vi "U8 Performance Test.vi"() -> ()   [LabVIEW 2021]
uses:
  ChannelCommon/typedef/Benchmark Stats.ctl
  ChannelCommon/typedef/Direction.ctl
  CIF_Iceoryx_PCAP_Universal.lvclass
  D:/dev/Packages/CIF_Channels_Core/src/CIFChannels/CIFChannels.lvclass
  Iceorxy Utilities/Typedef/PCAP Config.ctl
  ChannelCommon/typedef/New FIFO Config.ctl
  ChannelCommon/typedef/FIFO Flags.ctl
  Iceorxy Utilities/Typedef/PCAP Linktype.ctl
  ChannelCommon/typedef/New FIFO Instance Configuration.ctl
  <vilib>/Platform/TimedLoop/XDataNode/timing_clust.ctl
  <vilib>/Platform/TimedLoop/XDataNode/nitl_modes.ctl
  <vilib>/Platform/TimedLoop/XDataNode/wakeup.ctl
  ChannelCommon/typedef/TimeStamps.ctl
  CIFChannels/CIFChannels.lvclass/CIFChannels.ctl
  <vilib>/CIF Foundation/CIF Utilities/Statistics/I64/Stats_I64_CIF_U.lvclass/Stats_I64_CIF_U.ctl
  <vilib>/CIF Foundation/CIF Utilities/Statistics/I64/Get Stats.vi
  <vilib>/Platform/TimedLoop/XDataNode/XDataNode.xnode
  <vilib>/Platform/TimedLoop/XDataNode/XDNodeRunTimeDep.lvlib
  ChannelCommon/ChannelCommon.lvlib
  CIFChannels/CIFChannels.lvclass
  Iceorxy Utilities/Iceoryx Channel Utilities.lvlib
panel:
  in  "stop":bool
  out "Flatten (us) TO":T1
  out "Channel R/W (us) TO":T1
  out "Flatten (us)":T1
  out "Channel R/W (us)":T1
  out "avg TO":dbl
  out "max TO":dbl
  out "timed out? 3":bool
  out "timed out?":bool
  out "avg channel":dbl
  out "max channel":dbl
  out "pass":bool
  out "error out":errorcluster
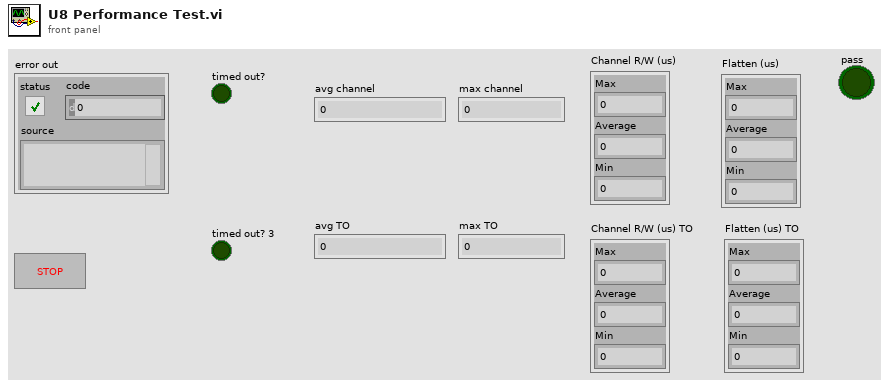
[diagram p1: front panel]
types:
  T1 = typedef "ChannelCommon.lvlib/Benchmark Stats.ctl" = cluster{"Max":i64, "Average":dbl, "Min":i64}
  T2 = typedef "Iceoryx Channel Utilities.lvlib/PCAP Config.ctl" = cluster{"New FIFO Config":T3, "Linktype":T5, "Linktype Override":u32, "Type Name Override":string}
  T3 = typedef "ChannelCommon.lvlib/New FIFO Config.ctl" = cluster{"Max Bytes/Msg":u64, "Max Msg/FIFO":u64, "FIFO Flags":T4, "Best Effort Subscribers":u32, "Backpressure Subscribers":u32}
  T4 = typedef "ChannelCommon.lvlib/FIFO Flags.ctl" = cluster{"Backpressure":bool, "Extended Config":bool}
  T5 = typedef "Iceoryx Channel Utilities.lvlib/PCAP Linktype.ctl" = u32
  T6 = typedef "ChannelCommon.lvlib/Direction.ctl" = enum8{"Publisher", "Subscriber"}
  T7 = typedef "ChannelCommon.lvlib/New FIFO Instance Configuration.ctl" = cluster{"Backpressure":bool, "Bytes/Message Override":u32, "Messages/FIFO Override":u32, "Custom Data":u8[]}
  T8 = typedef "ChannelCommon.lvlib/TimeStamps.ctl" = cluster{"ClockID":u8, "T0":i64, "T_Out":i64}
  T9 = typedef "XDNodeRunTimeDep.lvlib/timing_clust.ctl" = cluster{"Expected End [f-1]":u64, "Actual End [f-1]":u64, "Finished Late? [f-1]":bool, "Expected End [i-1]":u64, "Actual End [i-1]":u64, "Finished Late? [i-1]":bool, "Expected Start [i]":u64, "Actual Start [i]":u64, "Expected Start [f]":u64, "Actual Start [f]":u64, "Source Name":string, "Structure Name":string, "Period":i64, "Deadline":i64, "Offset":i64, "Start":i64, "Priority":i32, "Timeout":i32, "Mode":T10, "Wakeup Reason":T11, "Error":errorcluster, "Source Type":string, "Secondary Source Type":string, "Global End Time":u64, "Global Start Time":u64, "Frame Duration":u64, "Iteration Duration":u64, "Assigned CPU":i32, "I/O Scan Engine Mode":u32}
  T10 = typedef "XDNodeRunTimeDep.lvlib/nitl_modes.ctl" = enum32{"No Change", "Process missed periods, maintain original phase", "Discard missed periods, maintain original phase", "Process missed periods, ignore original phase", "Discard missed periods, ignore original phase"}
  T11 = typedef "XDNodeRunTimeDep.lvlib/wakeup.ctl" = enum32{"Normal", "Aborted", "Asynchronous wakeup", "Timing source error", "Timed loop error", "Timeout"}
  T12 = typedef "ChannelCommon.lvlib/New FIFO Instance Response.ctl" = cluster{"Publisher":string, "Custom Data":u8[]}
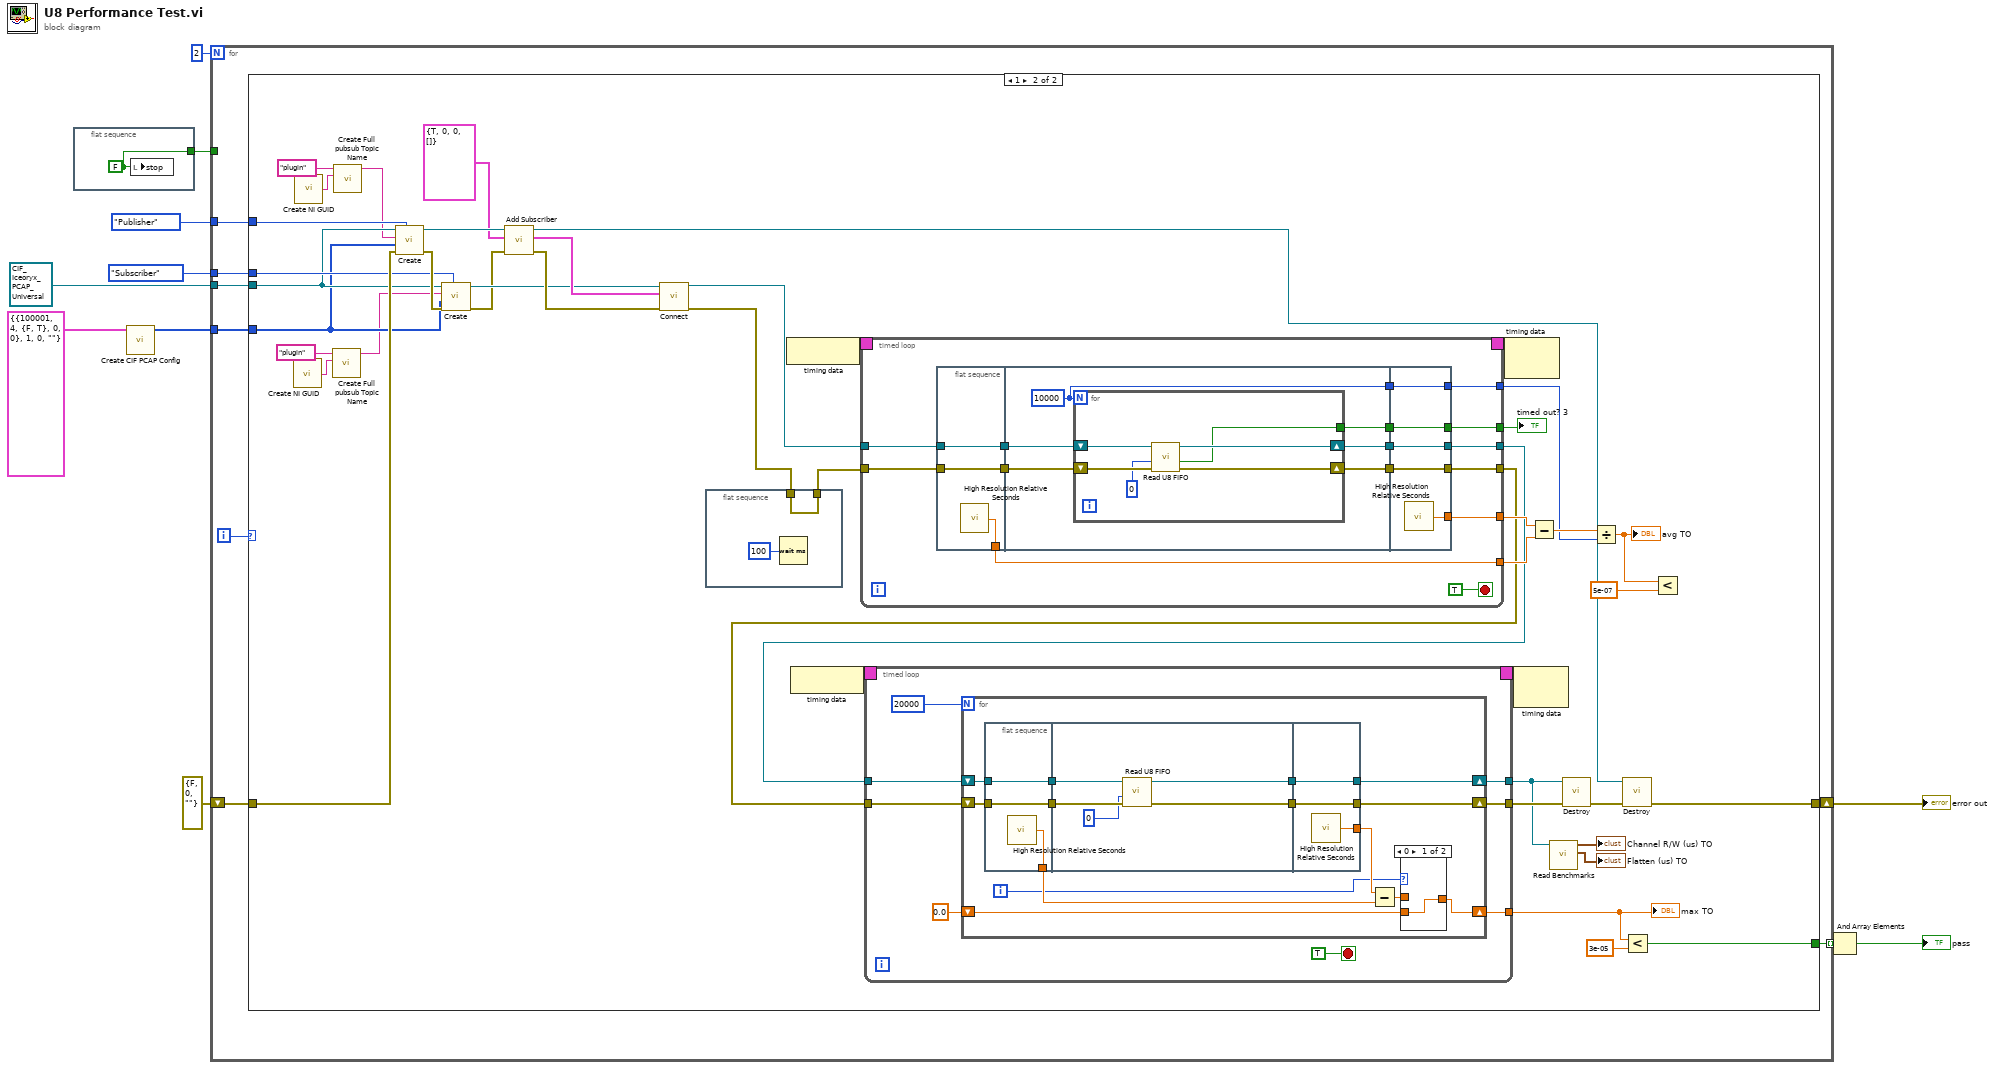
[diagram p0: block diagram]
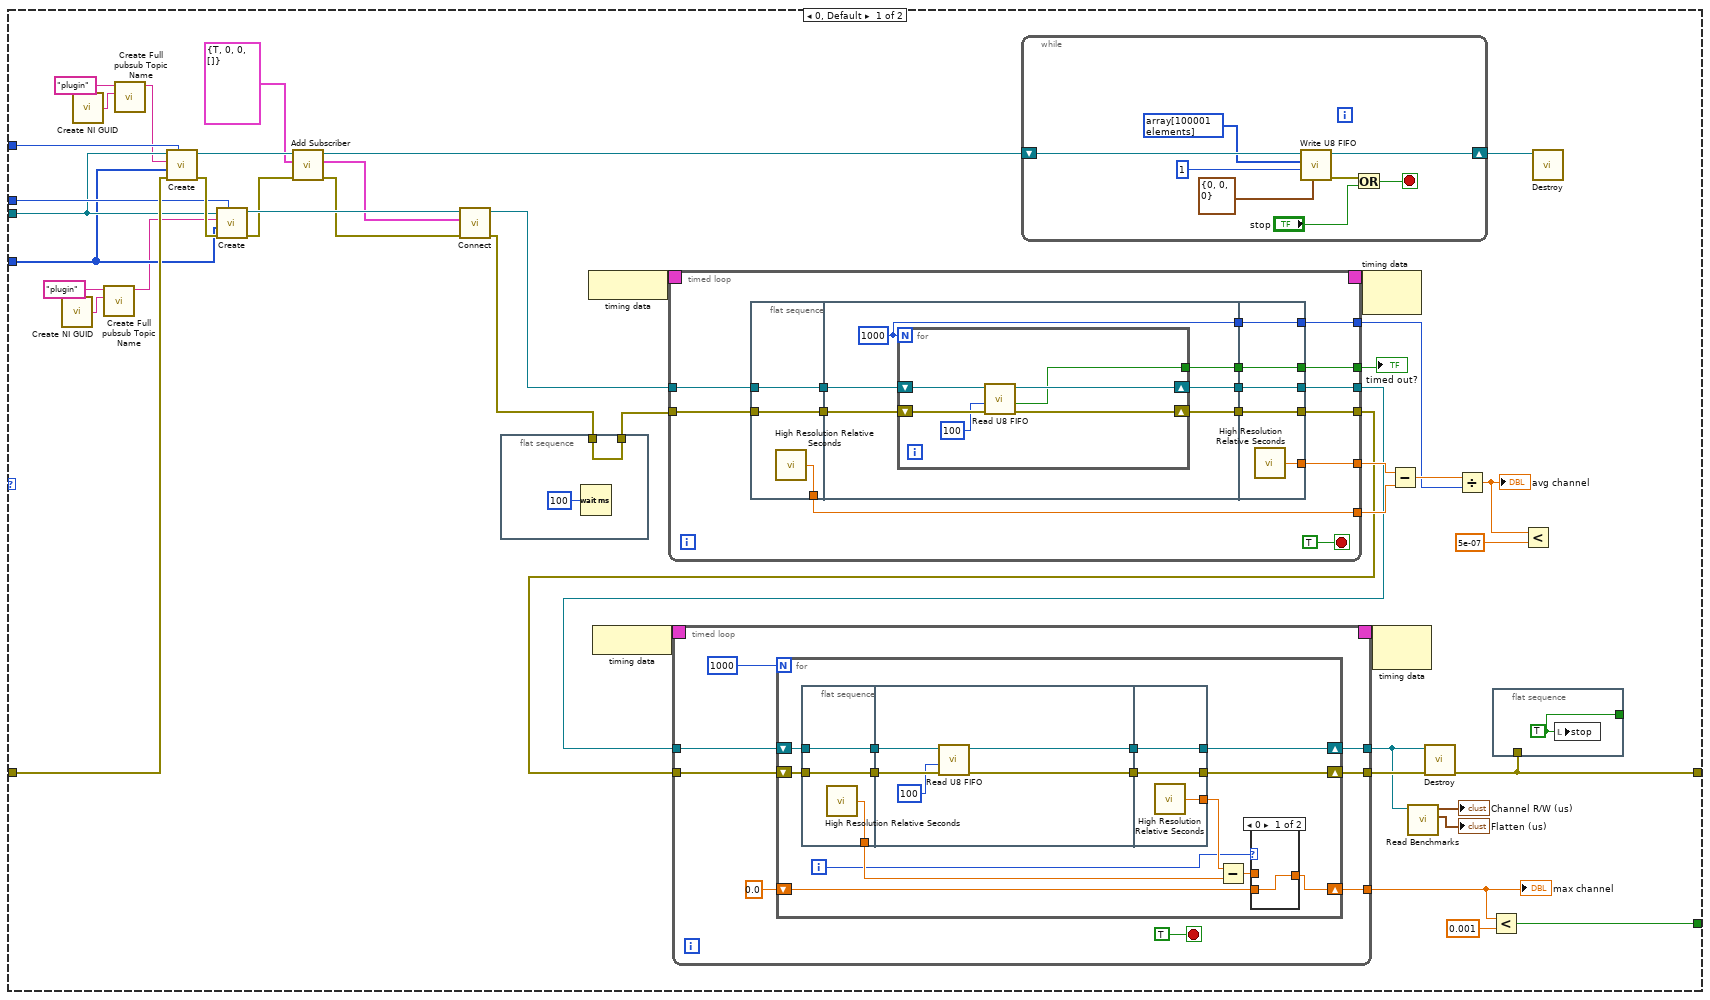
[diagram p2: hidden frame]
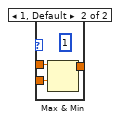
[diagram p3: hidden frame]
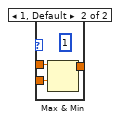
[diagram p4: hidden frame]
diagram:
  n1 = flat-sequence {
    tunnel: [w12] -> w3
    frame #0 {
      w12 = FALSE ("stop")
      n2 = local write "stop"(w12) -> ()
    }
  }
  n3 = call "Create CIF PCAP Config.vi"("PCAP FIFO Config"=T2 {"New FIFO Config"={"Max Bytes/Msg"=100001, "Max Msg/FIFO"=4, "FIFO Flags"={"Backpressure"=FALSE, "Extended Config"=TRUE}, "Best Effort Subscribers"=0, "Backpressure Subscribers"=0}, "Linktype"=1, "Linktype Override"=0, "Type Name Override"=""}) -> ("Flattened PCAP FIFO Config"=w1:u8[])  [unwired: 10 in]
  n4 = for {
    N: 2 -> [_]
    tunnel: [w20] -> w9 mode=indexing
    shift-right: [w19] -> w11
    shift-left: errorcluster {"status"=FALSE, "code"=0, "source"=""} ("error out") -> [w17]
    tunnel: Direction."Publisher" ("Direction") -> [w16]
    tunnel: Direction."Subscriber" ("Direction") -> [w15]
    tunnel: refnum<class "CIF_Iceoryx_PCAP_Universal.lvclass"> refnum ("CIF_CIPC_Fifo_U8.lvclass") -> [w14]
    tunnel: w1 -> [w13]
    tunnel: w3 -> [_]
    i -> [w18]
    n5 = case shown="1" w18 {
      tunnel: [w50 w185] -> w20
      tunnel: [w33 w176] -> w19
      tunnel: w17 -> [w48 w183]
      tunnel: w16 -> [w47 w182]
      tunnel: w15 -> [w46 w181]
      tunnel: w14 -> [w45 w180]
      tunnel: w13 -> [w43 w179]
      frame 0, Default {
        n6 = call <vilib>:"Create NI GUID.vi"() -> ("NI GUID"=w22:string)
        n7 = call <vilib>:"Create NI GUID.vi"() -> ("NI GUID"=w26:string)
        n8 = call "Create Full pubsub Topic Name.vi"("Topic"=w22, "Plugin name"="plugin") -> ("Full Topic"=w21:string)  [unwired: 8 in, 1 out]
        n9 = call "Create Full pubsub Topic Name.vi"("Topic"=w26, "Plugin name"="plugin") -> ("Full Topic"=w24:string)  [unwired: 8 in, 1 out]
        n10 = call-dynamic "Create.vi"("Direction"=w47, "error in (no error)"=w48, "Custom Config Data"=w43, "Name"=w24, "CIFFIFO in"=w45) -> ("error out"=w49:errorcluster, "CIFFIFO out"=w32:refnum<class "CIF_Iceoryx_PCAP_Universal.lvclass">)  [unwired: 5 in]
        n11 = call-dynamic "Create.vi"("Direction"=w46, "error in (no error)"=w49, "Custom Config Data"=w43, "Name"=w21, "CIFFIFO in"=w45) -> ("error out"=w30:errorcluster, "CIFFIFO out"=w44:refnum<class "CIF_Iceoryx_PCAP_Universal.lvclass">)  [unwired: 5 in]
        n12 = call-dynamic "Add Subscriber.vi"("error in (no error)"=w30, "New FIFO Instance Config"=T7 {"Backpressure"=TRUE, "Bytes/Message Override"=0, "Messages/FIFO Override"=0, "Custom Data"=[]}, "CIF_CIPC_Chn in"=w32) -> ("error out"=w29:errorcluster, "New FIFO Instance"=w28:T12, "CIF_CIPC_Chn out"=w31:refnum<class "CIF_Iceoryx_PCAP_Universal.lvclass">)  [unwired: 6 in]
        n13 = call-dynamic "Connect.vi"("error in (no error)"=w29, "Connection"=w28, "CIF_Iceoryx_PCAP"=w44) -> ("error out"=w40:errorcluster, "CIF_Iceoryx_PCAP"=w42:refnum<class "CIF_Iceoryx_PCAP_Universal.lvclass">)  [unwired: 7 in]
        n14 = flat-sequence {
          tunnel: w40 -> [w67]
          tunnel: [w67] -> w39
          frame #0 {
            n15 = Wait (ms)(milliseconds to wait=u32 100) -> ()  [unwired: 1 out]
          }
        }
        n16 = node-c288() -> (w64:T9)
        n17 = node-c288() -> (w62:T9)
        n18 = timed-loop {
          timing: w64 -> [_]
          timing-out: [_] -> w63
          tunnel: w42 -> [w131]
          tunnel: w39 -> [w130]
          tunnel: [w126] -> w56
          tunnel: [w124] -> w55
          tunnel: [w122] -> w60
          tunnel: [w121] -> w59
          tunnel: [w120] -> w57
          tunnel: [w118] -> w38
          stop <- TRUE stop-if-true
          n19 = flat-sequence {
            tunnel: w130 -> [w133]
            tunnel: w131 -> [w134]
            tunnel: [w134] -> w128
            tunnel: [w133] -> w127
            tunnel: [w132] -> w121
            tunnel: w128 -> [w140]
            tunnel: w127 -> [w139]
            tunnel: [w138] -> w125
            tunnel: [w137] -> w123
            tunnel: [w136] -> w119
            tunnel: [w135] -> w117
            tunnel: [w151] -> w126
            tunnel: w125 -> [w151]
            tunnel: [w150] -> w124
            tunnel: w123 -> [w150]
            tunnel: [w149] -> w122
            tunnel: [w148] -> w120
            tunnel: w119 -> [w148]
            tunnel: [w147] -> w118
            tunnel: w117 -> [w147]
            frame #0 {
              n20 = call <vilib>:"High Resolution Relative Seconds.vi"() -> ("relative seconds"=w132:dbl)
            }
            frame #1 {
              w136 = 1000
              n21 = for {
                N: w136 -> [_]
                shift-right: [w143] -> w138
                shift-left: w140 -> [w146]
                shift-right: [w144] -> w137
                shift-left: w139 -> [w145]
                tunnel: [w141] -> w135
                n22 = call-dynamic "Read U8 FIFO.vi"("error in (no error)"=w145, "Timeout (ms)"=100, "CIFFIFO in"=w146) -> ("error out"=w144:errorcluster, "timed out?"=w141:bool, "CIFFIFO out"=w143:refnum<class "CIF_Iceoryx_PCAP_Universal.lvclass">)  [unwired: 4 in, 2 out]
              }
            }
            frame #2 {
              n23 = call <vilib>:"High Resolution Relative Seconds.vi"() -> ("relative seconds"=w149:dbl)
            }
          }
        }
        "timed out?" <- w38
        n24 = timed-loop {
          timing: w62 -> [_]
          timing-out: [_] -> w61
          tunnel: w56 -> [w83]
          tunnel: w55 -> [w82]
          tunnel: [w80] -> w37
          tunnel: [w79] -> w41
          tunnel: [w76] -> w52
          stop <- TRUE stop-if-true
          n25 = for {
            N: 1000 -> [_]
            shift-right: [w92] -> w80
            shift-left: w83 -> [w94]
            shift-right: [w91] -> w79
            shift-left: w82 -> [w93]
            shift-right: [w86] -> w76
            shift-left: 0.0 -> [w87]
            i -> [w85]
            n26 = flat-sequence {
              tunnel: w93 -> [w103]
              tunnel: w94 -> [w104]
              tunnel: [w104] -> w97
              tunnel: [w103] -> w96
              tunnel: [w102] -> w89
              tunnel: w97 -> [w109]
              tunnel: w96 -> [w108]
              tunnel: [w106] -> w95
              tunnel: [w107] -> w84
              tunnel: [w112] -> w92
              tunnel: w95 -> [w112]
              tunnel: [w111] -> w91
              tunnel: [w110] -> w90
              tunnel: w84 -> [w111]
              frame #0 {
                n27 = call <vilib>:"High Resolution Relative Seconds.vi"() -> ("relative seconds"=w102:dbl)
              }
              frame #1 {
                n28 = call-dynamic "Read U8 FIFO.vi"("error in (no error)"=w108, "Timeout (ms)"=100, "CIFFIFO in"=w109) -> ("error out"=w107:errorcluster, "CIFFIFO out"=w106:refnum<class "CIF_Iceoryx_PCAP_Universal.lvclass">)  [unwired: 4 in, 3 out]
              }
              frame #2 {
                n29 = call <vilib>:"High Resolution Relative Seconds.vi"() -> ("relative seconds"=w110:dbl)
              }
            }
            n30 = Subtract(x=w90, y=w89) -> (x-y=w88:dbl)
            n31 = case shown="0" w85 {
              tunnel: w88 -> [_ w101]
              tunnel: w87 -> [w98 w100]
              tunnel: [w98 w99] -> w86
              frame 0 {
              }
              frame 1, Default {
                (unwired) u32 1 ("milliseconds to wait")
                n32 = Max & Min(x=w101, y=w100) -> (max(x,y)=w99:dbl)  [unwired: 1 out]
              }
            }
          }
        }
        "max channel" <- w52
        n33 = while {
          shift-right: [w73] -> w34
          shift-left: w31 -> [w75]
          stop <- w70 stop-if-true
          n34 = call-dynamic "Write U8 FIFO.vi"("FIFO Timestamps"=T8 {"ClockID"=0, "T0"=0, "T_Out"=0}, "Timeout (ms)"=1, "Data in"=u8[] array[100001 elements] ("U8 Data"), "CIFFIFO in"=w75) -> ("error out"=w71:errorcluster, "CIFFIFO out"=w73:refnum<class "CIF_Iceoryx_PCAP_Universal.lvclass">)  [unwired: 4 in, 2 out]
          n35 = Or(x=w71, y="stop") -> (x .or. y?=w70:bool)
        }
        n36 = node-c288(w63) -> ()  [unwired: 1 out]
        n37 = node-c288(w61) -> ()  [unwired: 1 out]
        n38 = Subtract(x=w60, y=w59) -> (x-y=w58:dbl)
        n39 = call "Read Benchmarks.vi"("CIFChannels in"=w37) -> ("Flatten (us)"=→"Flatten (us)":T1, "Channel R/W (us)"=→"Channel R/W (us)":T1)  [unwired: 9 in]
        n40 = call-dynamic "Destroy.vi"("error in (no error)"=w41, "Icoryx_PCAP in"=w37) -> ("error out"=w33:errorcluster)  [unwired: 8 in, 1 out]
        n41 = Divide(x=w58, y=w57) -> (x/y=w54:dbl)
        "avg channel" <- w54
        n42 = Less?(x=w52, y=0.001) -> (x < y?=w50:bool)
        n43 = flat-sequence {
          tunnel: [w65] -> _
          tunnel: w33 -> [_]
          frame #0 {
            w65 = TRUE ("stop")
            n44 = local write "stop"(w65) -> ()
          }
        }
        n45 = Less?(x=w54, y=5e-07) -> ()  [unwired: 1 out]
        n46 = call-dynamic "Destroy.vi"("Icoryx_PCAP in"=w34) -> ()  [unwired: 9 in, 2 out]
      }
      frame 1 {
        n47 = call <vilib>:"Create NI GUID.vi"() -> ("NI GUID"=w157:string)
        n48 = call <vilib>:"Create NI GUID.vi"() -> ("NI GUID"=w161:string)
        n49 = call "Create Full pubsub Topic Name.vi"("Topic"=w157, "Plugin name"="plugin") -> ("Full Topic"=w156:string)  [unwired: 8 in, 1 out]
        n50 = call "Create Full pubsub Topic Name.vi"("Topic"=w161, "Plugin name"="plugin") -> ("Full Topic"=w159:string)  [unwired: 8 in, 1 out]
        n51 = call-dynamic "Create.vi"("Direction"=w182, "error in (no error)"=w183, "Custom Config Data"=w179, "Name"=w159, "CIFFIFO in"=w180) -> ("error out"=w184:errorcluster, "CIFFIFO out"=w167:refnum<class "CIF_Iceoryx_PCAP_Universal.lvclass">)  [unwired: 5 in]
        n52 = call-dynamic "Create.vi"("Direction"=w181, "error in (no error)"=w184, "Custom Config Data"=w179, "Name"=w156, "CIFFIFO in"=w180) -> ("error out"=w166:errorcluster, "CIFFIFO out"=w168:refnum<class "CIF_Iceoryx_PCAP_Universal.lvclass">)  [unwired: 5 in]
        n53 = call-dynamic "Add Subscriber.vi"("error in (no error)"=w166, "New FIFO Instance Config"=T7 {"Backpressure"=TRUE, "Bytes/Message Override"=0, "Messages/FIFO Override"=0, "Custom Data"=[]}, "CIF_CIPC_Chn in"=w167) -> ("error out"=w170:errorcluster, "New FIFO Instance"=w169:T12, "CIF_CIPC_Chn out"=w163:refnum<class "CIF_Iceoryx_PCAP_Universal.lvclass">)  [unwired: 6 in]
        n54 = call-dynamic "Connect.vi"("error in (no error)"=w170, "Connection"=w169, "CIF_Iceoryx_PCAP"=w168) -> ("error out"=w165:errorcluster, "CIF_Iceoryx_PCAP"=w164:refnum<class "CIF_Iceoryx_PCAP_Universal.lvclass">)  [unwired: 7 in]
        n55 = flat-sequence {
          tunnel: w165 -> [w201]
          tunnel: [w201] -> w175
          frame #0 {
            n56 = Wait (ms)(milliseconds to wait=u32 100) -> ()  [unwired: 1 out]
          }
        }
        n57 = node-c288() -> (w199:T9)
        n58 = node-c288() -> (w197:T9)
        n59 = timed-loop {
          timing: w199 -> [_]
          timing-out: [_] -> w198
          tunnel: w164 -> [w257]
          tunnel: w175 -> [w256]
          tunnel: [w252] -> w191
          tunnel: [w250] -> w190
          tunnel: [w248] -> w195
          tunnel: [w247] -> w194
          tunnel: [w246] -> w192
          tunnel: [w244] -> w174
          stop <- TRUE stop-if-true
          n60 = flat-sequence {
            tunnel: w256 -> [w259]
            tunnel: w257 -> [w260]
            tunnel: [w260] -> w254
            tunnel: [w259] -> w253
            tunnel: [w258] -> w247
            tunnel: w254 -> [w266]
            tunnel: w253 -> [w265]
            tunnel: [w264] -> w251
            tunnel: [w263] -> w249
            tunnel: [w262] -> w245
            tunnel: [w261] -> w243
            tunnel: [w277] -> w252
            tunnel: w251 -> [w277]
            tunnel: [w276] -> w250
            tunnel: w249 -> [w276]
            tunnel: [w275] -> w248
            tunnel: [w274] -> w246
            tunnel: w245 -> [w274]
            tunnel: [w273] -> w244
            tunnel: w243 -> [w273]
            frame #0 {
              n61 = call <vilib>:"High Resolution Relative Seconds.vi"() -> ("relative seconds"=w258:dbl)
            }
            frame #1 {
              w262 = 10000
              n62 = for {
                N: w262 -> [_]
                shift-right: [w269] -> w264
                shift-left: w266 -> [w272]
                shift-right: [w270] -> w263
                shift-left: w265 -> [w271]
                tunnel: [w268] -> w261
                n63 = call-dynamic "Read U8 FIFO.vi"("error in (no error)"=w271, "Timeout (ms)"=0, "CIFFIFO in"=w272) -> ("error out"=w270:errorcluster, "timed out?"=w268:bool, "CIFFIFO out"=w269:refnum<class "CIF_Iceoryx_PCAP_Universal.lvclass">)  [unwired: 4 in, 2 out]
              }
            }
            frame #2 {
              n64 = call <vilib>:"High Resolution Relative Seconds.vi"() -> ("relative seconds"=w275:dbl)
            }
          }
        }
        "timed out? 3" <- w174
        n65 = timed-loop {
          timing: w197 -> [_]
          timing-out: [_] -> w196
          tunnel: w191 -> [w209]
          tunnel: w190 -> [w208]
          tunnel: [w206] -> w171
          tunnel: [w205] -> w178
          tunnel: [w202] -> w187
          stop <- TRUE stop-if-true
          n66 = for {
            N: 20000 -> [_]
            shift-right: [w218] -> w206
            shift-left: w209 -> [w220]
            shift-right: [w217] -> w205
            shift-left: w208 -> [w219]
            shift-right: [w212] -> w202
            shift-left: 0.0 -> [w213]
            i -> [w211]
            n67 = flat-sequence {
              tunnel: w219 -> [w229]
              tunnel: w220 -> [w230]
              tunnel: [w230] -> w223
              tunnel: [w229] -> w222
              tunnel: [w228] -> w215
              tunnel: w223 -> [w235]
              tunnel: w222 -> [w233]
              tunnel: [w234] -> w221
              tunnel: [w232] -> w210
              tunnel: [w238] -> w218
              tunnel: w221 -> [w238]
              tunnel: [w237] -> w217
              tunnel: [w236] -> w216
              tunnel: w210 -> [w237]
              frame #0 {
                n68 = call <vilib>:"High Resolution Relative Seconds.vi"() -> ("relative seconds"=w228:dbl)
              }
              frame #1 {
                n69 = call-dynamic "Read U8 FIFO.vi"("error in (no error)"=w233, "Timeout (ms)"=0, "CIFFIFO in"=w235) -> ("error out"=w232:errorcluster, "CIFFIFO out"=w234:refnum<class "CIF_Iceoryx_PCAP_Universal.lvclass">)  [unwired: 4 in, 3 out]
              }
              frame #2 {
                n70 = call <vilib>:"High Resolution Relative Seconds.vi"() -> ("relative seconds"=w236:dbl)
              }
            }
            n71 = Subtract(x=w216, y=w215) -> (x-y=w214:dbl)
            n72 = case shown="0" w211 {
              tunnel: w214 -> [_ w227]
              tunnel: w213 -> [w224 w226]
              tunnel: [w224 w225] -> w212
              frame 0 {
              }
              frame 1, Default {
                (unwired) u32 1 ("milliseconds to wait")
                n73 = Max & Min(x=w227, y=w226) -> (max(x,y)=w225:dbl)  [unwired: 1 out]
              }
            }
          }
        }
        "max TO" <- w187
        n74 = node-c288(w198) -> ()  [unwired: 1 out]
        n75 = node-c288(w196) -> ()  [unwired: 1 out]
        n76 = Subtract(x=w195, y=w194) -> (x-y=w193:dbl)
        n77 = call "Read Benchmarks.vi"("CIFChannels in"=w171) -> ("Flatten (us)"=→"Flatten (us) TO":T1, "Channel R/W (us)"=→"Channel R/W (us) TO":T1)  [unwired: 9 in]
        n78 = call-dynamic "Destroy.vi"("error in (no error)"=w178, "Icoryx_PCAP in"=w171) -> ("error out"=w177:errorcluster)  [unwired: 8 in, 1 out]
        n79 = Divide(x=w193, y=w192) -> (x/y=w189:dbl)
        "avg TO" <- w189
        n80 = call-dynamic "Destroy.vi"("error in (no error)"=w177, "Icoryx_PCAP in"=w163) -> ("error out"=w176:errorcluster)  [unwired: 8 in, 1 out]
        n81 = Less?(x=w187, y=3e-05) -> (x < y?=w185:bool)
        n82 = Less?(x=w189, y=5e-07) -> ()  [unwired: 1 out]
      }
    }
  }
  "error out" <- w11
  n83 = And Array Elements(Boolean array=w9) -> (logical AND=→"pass":bool)
